vi "LoadCfgFromFile.vi"(8 "error in (no error)":errorcluster, 10 "Configuration FIle":path, 11 "object in":refnum<class "Channel.lvclass">) -> (0 "error out":errorcluster, 2 "Success?":bool, 3 "object out":refnum<class "Channel.lvclass">)   [LabVIEW 2021, in "Channel.lvlib" / "Channel.lvclass"]
doc: "Reads the Ini file and loads the Configuration"
uses:
  Channel.lvclass
  Configuration_class/properties/WriteConfigurationFile.vi
  Configuration_class/Configuration.lvclass
  Channel.lvclass/Channel.ctl
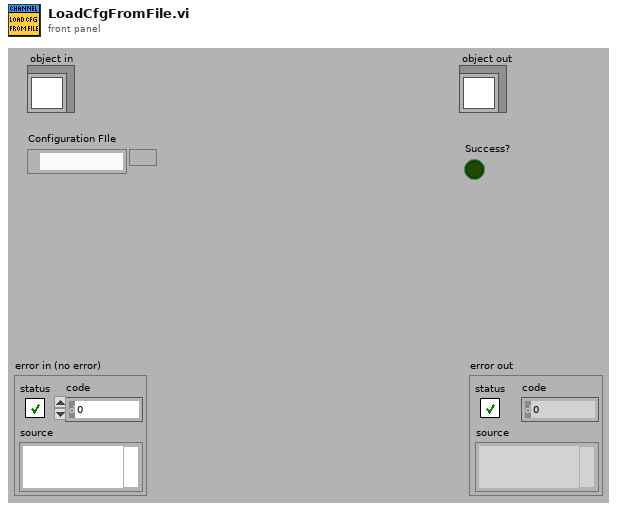
[diagram p1: front panel]
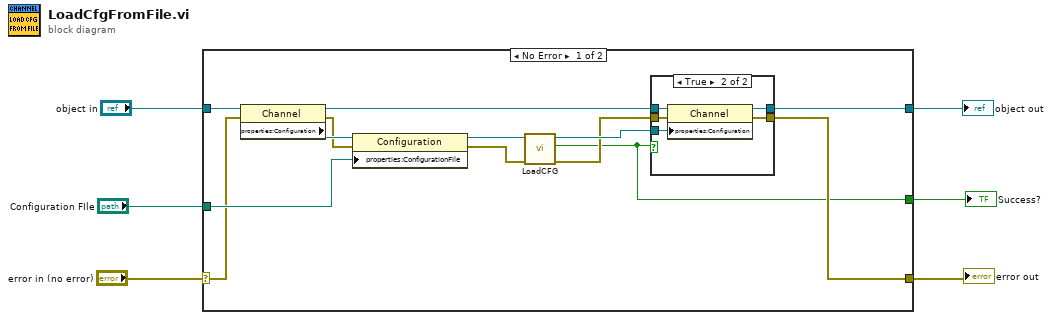
[diagram p0: block diagram]
diagram:
  n1 = case shown="No Error" "error in (no error)" {
    selector: "error in (no error)" -> [w14 w28]
    tunnel: [w8 w28] -> w5
    tunnel: [w13 w27] -> w3
    tunnel: "object in" -> [w19 w27]
    tunnel: "Configuration FIle" -> [w16 _]
    tunnel: [w7 _] -> w1
    frame No Error {
      n2 = property class="Channel"(reference=w19, error in=w14) -> (reference out=w18:refnum<class "Channel.lvclass">, error out=w15:errorcluster, "properties:Configuration"=w17:refnum<class "Configuration.lvclass">)
      n3 = property class="Configuration"(reference=w17, error in=w15, "properties:ConfigurationFile"=w16) -> (reference out=w12:refnum<class "Configuration.lvclass">, error out=w10:errorcluster)
      n4 = call-dynamic "LoadCFG.vi"("error in (no error)"=w10, "object in"=w12) -> ("error out"=w9:errorcluster, "Success?"=w7:bool, "object out"=w11:refnum<class "Configuration.lvclass">)  [unwired: 7 in]
      n5 = case shown="True" w7 {
        tunnel: w18 -> [w21 w26]
        tunnel: [w21 w25] -> w13
        tunnel: w11 -> [_ w24]
        tunnel: w9 -> [w20 w23]
        tunnel: [w20 w22] -> w8
        frame False {
        }
        frame True {
          n6 = property class="Channel"(reference=w26, error in=w23, "properties:Configuration"=w24) -> (reference out=w25:refnum<class "Channel.lvclass">, error out=w22:errorcluster)
        }
      }
    }
    frame Error {
    }
  }
  "error out" <- w5
  "object out" <- w3
  "Success?" <- w1
